vi "Test Withdraw Funds.vi"() -> ()   [LabVIEW 2026]
doc: "Caraya unit test for Withdraw Funds.vi. Every case starts from its own fresh copy of the specification accounts file (Create Accounts Fixture.vi, written under Tests\\results), so the real ATM accounts.txt is never touched and the cases can run in parallel. The balance is always checked by reading the file back with Get Account.vi.\n\nCase 1: withdrawing 50 from 23456 (balance 1000) succeeds and the file holds 950.\nCase 2: withdrawing 800 from 34567 (balance 750) is refused (Sufficient Funds? FALSE) and the file still holds 750 - the exam's Withdrawal Failed path.\nCase 3: withdrawing the exact balance 550 from 12345 is allowed and leaves 0.\n\nThe error cluster carries the FIRST failure only. Read the JUnit report for all of them."
uses:
  <vilib>/addons/_JKI Toolkits/Caraya/classes/Test/Test.lvclass
  <vilib>/addons/_JKI Toolkits/Caraya/classes/Assert/Assert.lvclass
panel:
  out "error out":errorcluster
  in  "error in":errorcluster
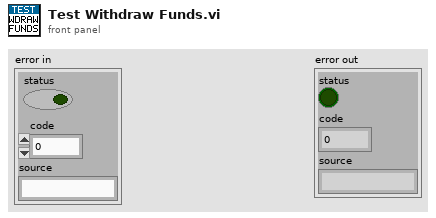
[diagram p1: front panel]
types:
  T1 = cluster{"Account Number":string, "First Name":string, "Last Name":string, "Balance":dbl}
  T2 = typedef "ATM Account.ctl" = cluster{"Account Number":string, "First Name":string, "Last Name":string, "Balance":dbl}
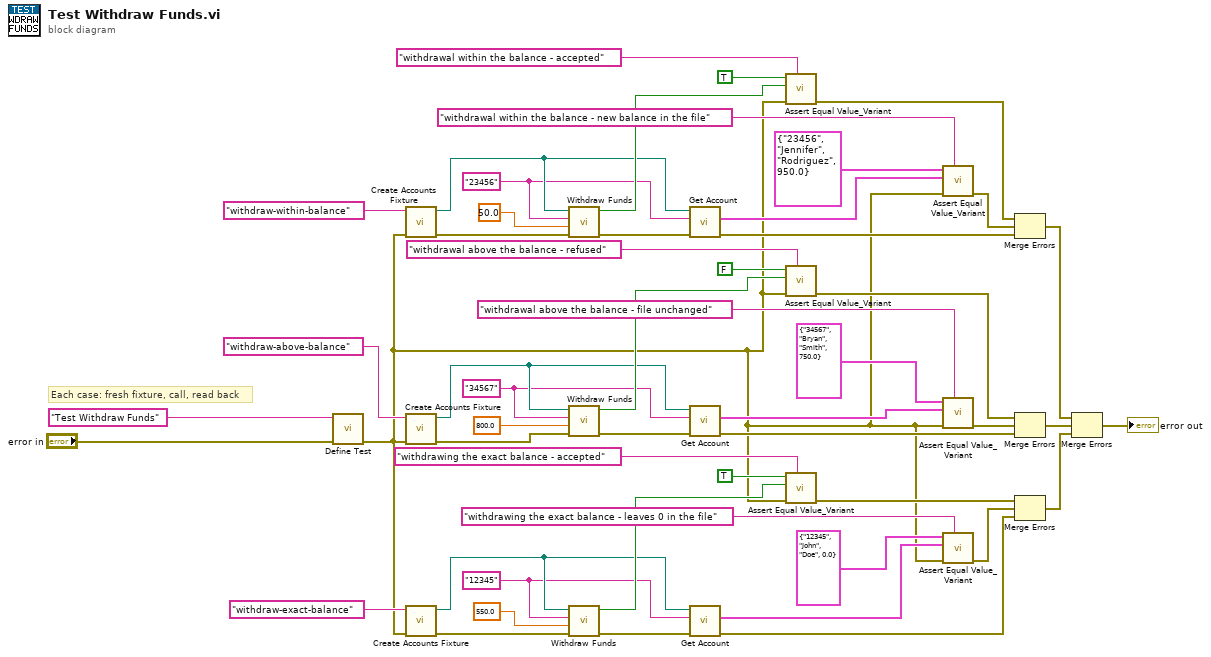
[diagram p0: block diagram]
diagram:
  w36 = "12345" ("Account Number")
  w21 = "34567" ("Account Number")
  w6 = "23456" ("Account Number")
  # "Each case: fresh fixture, call, read back"
  n1 = call <vilib>:"Define Test.vi"("error in (no error)"="error in", "Label (VI Title)"="Test Withdraw Funds") -> ("error out"=w4:errorcluster)  [unwired: 8 in, 1 out]
  n2 = call "Create Accounts Fixture.vi"("error in"=w4, "Fixture Name"="withdraw-within-balance") -> ("error out"=w9:errorcluster, "Accounts File Path"=w8:path)  [unwired: 8 in]
  n3 = call "Create Accounts Fixture.vi"("error in"=w4, "Fixture Name"="withdraw-above-balance") -> ("error out"=w24:errorcluster, "Accounts File Path"=w23:path)  [unwired: 8 in]
  n4 = call "Create Accounts Fixture.vi"("error in"=w4, "Fixture Name"="withdraw-exact-balance") -> ("error out"=w39:errorcluster, "Accounts File Path"=w38:path)  [unwired: 8 in]
  n5 = call "Withdraw Funds.vi"("error in"=w9, "Amount"=50.0, "Account Number"=w6, "Accounts File Path"=w8) -> ("error out"=w11:errorcluster, "Sufficient Funds?"=w10:bool)  [unwired: 5 in, 1 out]
  n6 = call "Withdraw Funds.vi"("error in"=w24, "Amount"=800.0, "Account Number"=w21, "Accounts File Path"=w23) -> ("error out"=w26:errorcluster, "Sufficient Funds?"=w25:bool)  [unwired: 5 in, 1 out]
  n7 = call "Withdraw Funds.vi"("error in"=w39, "Amount"=550.0, "Account Number"=w36, "Accounts File Path"=w38) -> ("error out"=w41:errorcluster, "Sufficient Funds?"=w40:bool)  [unwired: 5 in, 1 out]
  n8 = call "Get Account.vi"("error in"=w11, "Account Number"=w6, "Accounts File Path"=w8) -> ("error out"=w13:errorcluster, "Account"=w12:T2)  [unwired: 6 in, 1 out]
  n9 = call "Get Account.vi"("error in"=w26, "Account Number"=w21, "Accounts File Path"=w23) -> ("error out"=w28:errorcluster, "Account"=w27:T2)  [unwired: 6 in, 1 out]
  n10 = call "Get Account.vi"("error in"=w41, "Account Number"=w36, "Accounts File Path"=w38) -> ("error out"=w43:errorcluster, "Account"=w42:T2)  [unwired: 6 in, 1 out]
  n11 = call <vilib>:"Assert Equal Value_Variant.vi"("Label"="withdrawal within the balance - accepted", "error in (no error)"=w4, "Actual"=w10, "Expected"=TRUE ("expected 1")) -> ("error out"=w16:errorcluster)  [unwired: 6 in, 1 out]
  n12 = call <vilib>:"Assert Equal Value_Variant.vi"("Label"="withdrawal above the balance - refused", "error in (no error)"=w4, "Actual"=w25, "Expected"=FALSE ("expected 3")) -> ("error out"=w31:errorcluster)  [unwired: 6 in, 1 out]
  n13 = call <vilib>:"Assert Equal Value_Variant.vi"("Label"="withdrawing the exact balance - accepted", "error in (no error)"=w4, "Actual"=w40, "Expected"=TRUE ("expected 5")) -> ("error out"=w46:errorcluster)  [unwired: 6 in, 1 out]
  n14 = call <vilib>:"Assert Equal Value_Variant.vi"("Label"="withdrawal within the balance - new balance in the file", "error in (no error)"=w4, "Actual"=w12, "Expected"=T1 {"Account Number"="23456", "First Name"="Jennifer", "Last Name"="Rodriguez", "Balance"=950.0} ("expected 2")) -> ("error out"=w19:errorcluster)  [unwired: 6 in, 1 out]
  n15 = call <vilib>:"Assert Equal Value_Variant.vi"("Label"="withdrawal above the balance - file unchanged", "error in (no error)"=w4, "Actual"=w27, "Expected"=T1 {"Account Number"="34567", "First Name"="Bryan", "Last Name"="Smith", "Balance"=750.0} ("expected 4")) -> ("error out"=w34:errorcluster)  [unwired: 6 in, 1 out]
  n16 = call <vilib>:"Assert Equal Value_Variant.vi"("Label"="withdrawing the exact balance - leaves 0 in the file", "error in (no error)"=w4, "Actual"=w42, "Expected"=T1 {"Account Number"="12345", "First Name"="John", "Last Name"="Doe", "Balance"=0.0} ("expected 6")) -> ("error out"=w49:errorcluster)  [unwired: 6 in, 1 out]
  n17 = Merge Errors(w16, w19, w13) -> (w50:errorcluster)
  n18 = Merge Errors(w31, w34, w28) -> (w51:errorcluster)
  n19 = Merge Errors(w46, w49, w43) -> (w52:errorcluster)
  n20 = Merge Errors(w50, w51, w52) -> (→"error out":errorcluster)
